vi "DialogAddDesignPattern.vi"(0 "ClassWriterNative":refnum<class "ClassWriterNative.lvclass">, 1 "ClassItemRefIn":refnum<vi>, 5 "error in (no error)":errorcluster) -> (14 "ClassWriterNative":refnum<class "ClassWriterNative.lvclass">, 15 "ClassItemRefOut":refnum<vi>, 16 "AddDesignPatternData":T1, 17 "Cancelled":bool, 19 "error out":errorcluster)   [LabVIEW 2020, in "ClassWriterNative.lvclass"]
uses:
  ClassWriterNative.lvclass
  Provider_BaseClassInterface/AddDesignPatternData.ctl
  Provider_BaseClassInterface/DesignPatternsData.ctl
  Common/LvClass_class/GDSLvClass_PlugIn.ctl
  Common/LvClass_class/GDSLvClass_PlugInTypes.ctl
  Provider_BaseClassInterface/BaseProvider_SubVIs/BaseProvider_DesignPatternsActions.ctl
  ClassWriterNative.lvclass/ClassWriterNative.ctl
panel:
  out "ProductPicture":picture
  out "TextError":string
  out "_Description":string caption="Description"
  in  "_DesignPatterns":string(tree) caption="Design Patterns"
  out "_ClassTemplateUsed":string caption="Class Template Used"
  out "_ClassProviderName":string caption="Class Provider Name"
  out "_ClassName":string caption="Class name"
  in  "_ShowContextHelp":bool
  in  "Help":bool
  in  "_Cancel":bool
  in  "_Next":bool
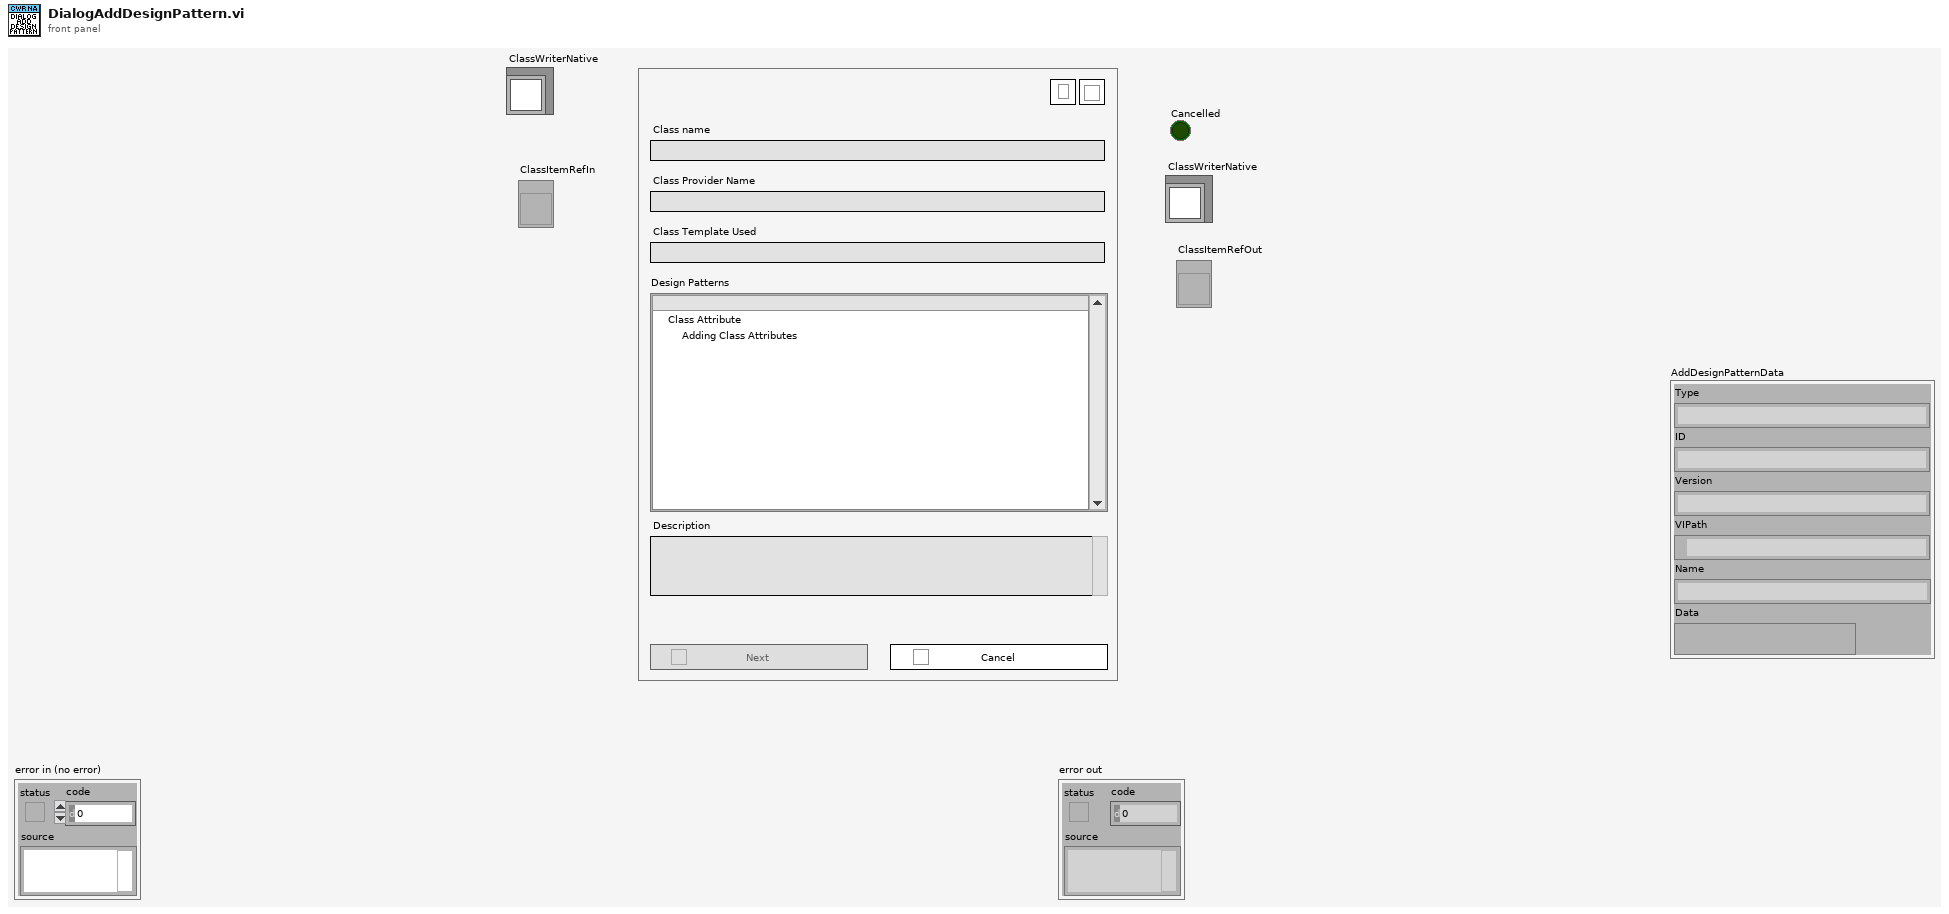
[diagram p1: front panel]
types:
  T1 = typedef "AddDesignPatternData.ctl" = cluster{"Type":string, "ID":string, "Version":string, "VIPath":path, "Name":string, "Data":variant}
  T2 = typedef "DesignPatternsData.ctl" = cluster{"Type":string, "Patterns":cluster{"ID":string, "Path":path, "Name":string, "Desc":string, "Version":string, "DependenciesID":string[], "OnlyOne":bool}[]}
  T3 = cluster{"Cancel":bool, "ClassProviderName":string, "ClassTemplateUsed":string, "DesignPatterns":T2[], "DataOut":variant, "PlugInVI":path, "DesignPatternID":string, "DesignPatternType":string, "PlugInIDs":string[], "DesignPatternVer":string, "Name":string}
  T4 = typedef "BaseProvider_DesignPatternsActions.ctl" = enum16{"AddPatternDialog", "GeneratePattern", "RemovePattern", "CreatePatternMethod", "UpdatePattern"}
  T5 = typedef "GDSLvClass_PlugIn.ctl" = cluster{"Type":T6, "ID":string, "Version":string, "Path":path, "Name":string, "Data":variant}
  T6 = typedef "GDSLvClass_PlugInTypes.ctl" = enum16{"DesignPattern", "MethodTypes"}
  T7 = typedef "GDSLvCLass_ClassSettingsType.ctl" = cluster{"ClassProviderName":string, "ClassTemplateUsed":string, "ClassTemplateVersion":string, "ClassDescription":string, "PlugIns":T5[], "ConnectorPanePattern":string}
  T8 = cluster{"ID":string, "Path":path, "Name":string, "Desc":string, "Version":string, "DependenciesID":string[], "OnlyOne":bool}[]
  T9 = cluster{"ID":string, "Path":path, "Name":string, "Desc":string, "Version":string, "DependenciesID":string[], "OnlyOne":bool}
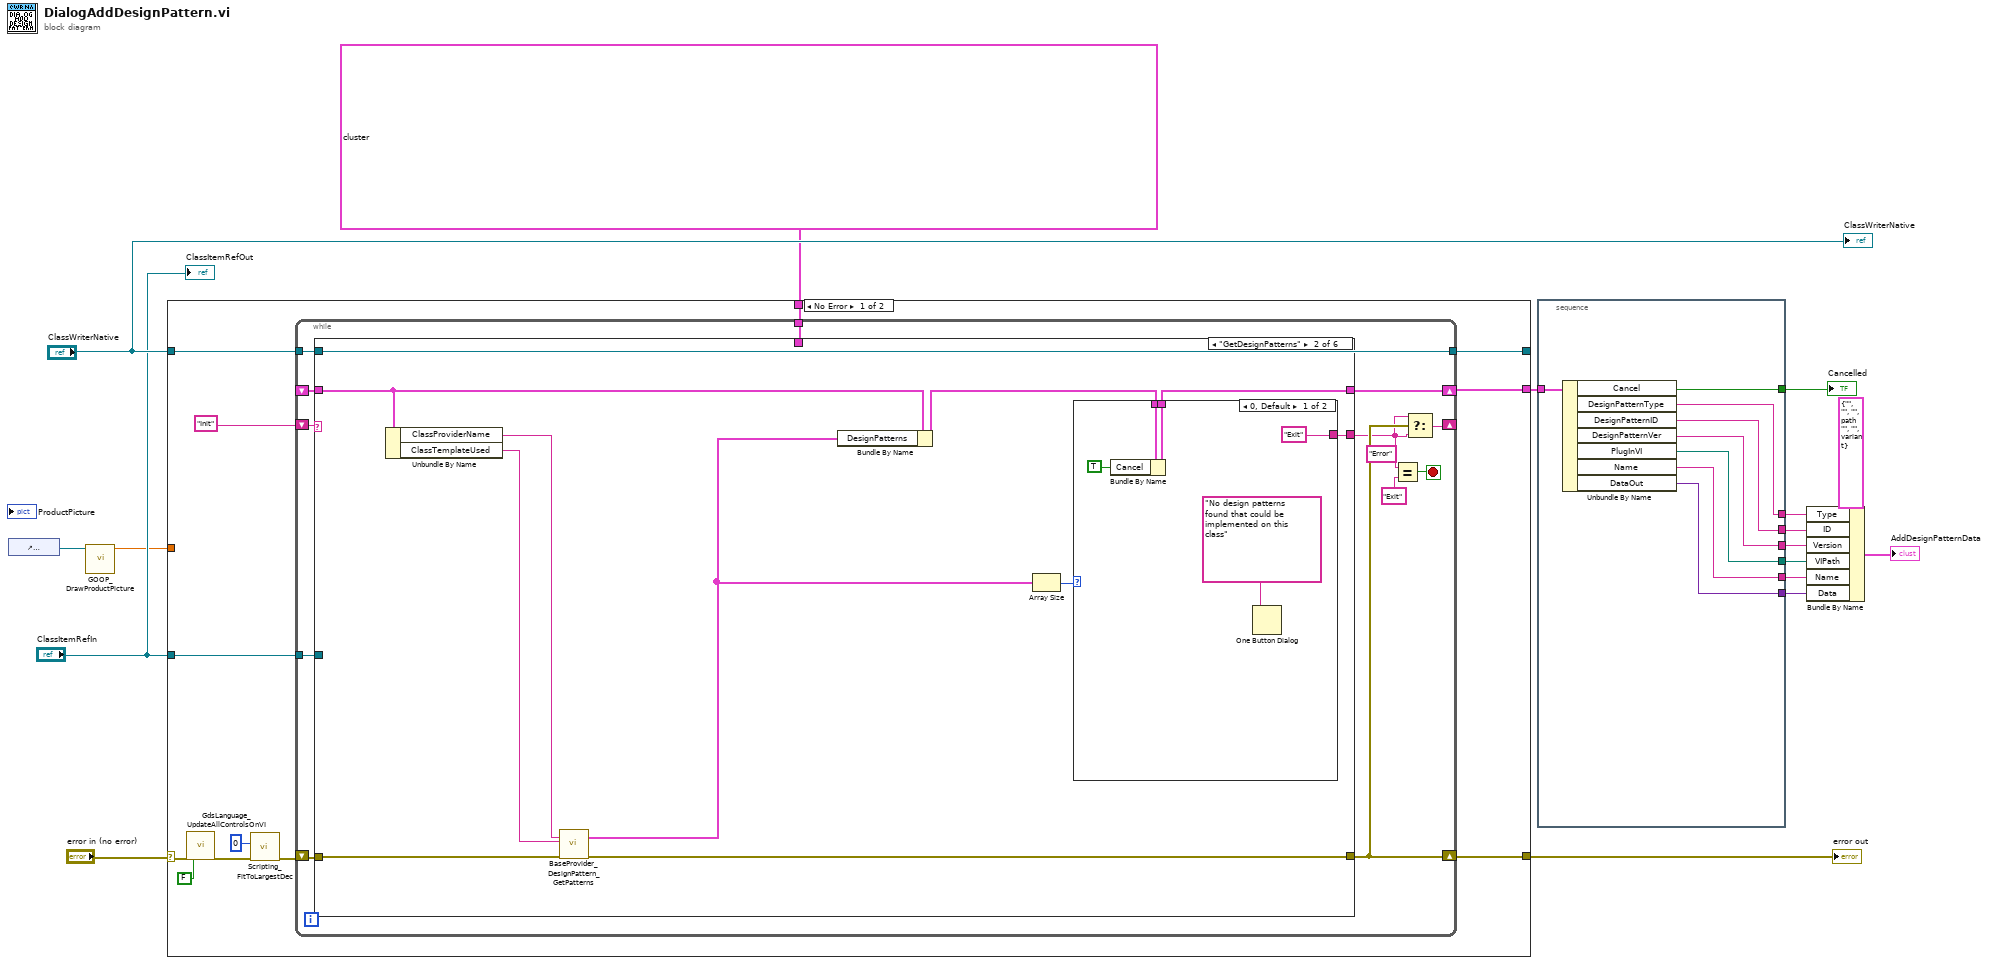
[diagram p0: block diagram]
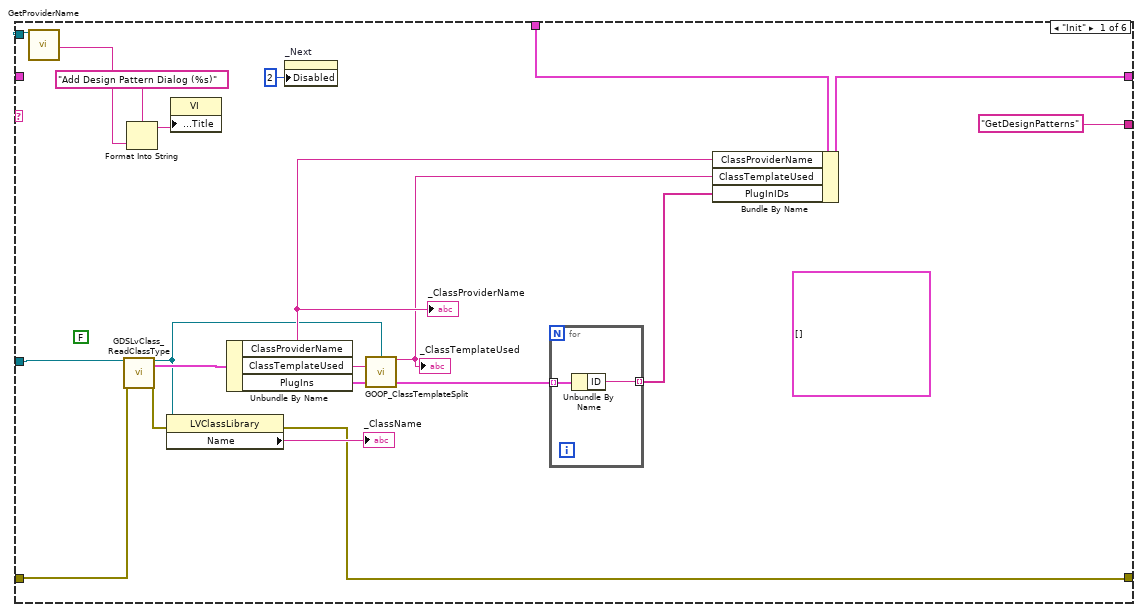
[diagram p2: hidden frame]
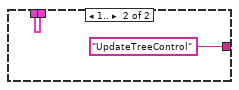
[diagram p3: hidden frame]
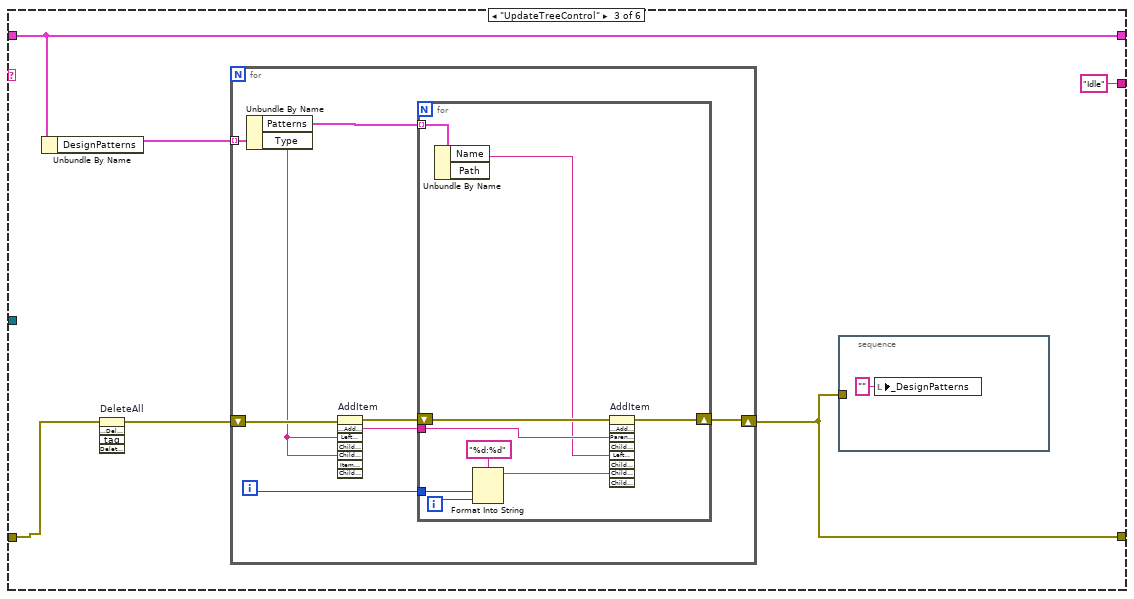
[diagram p4: hidden frame]
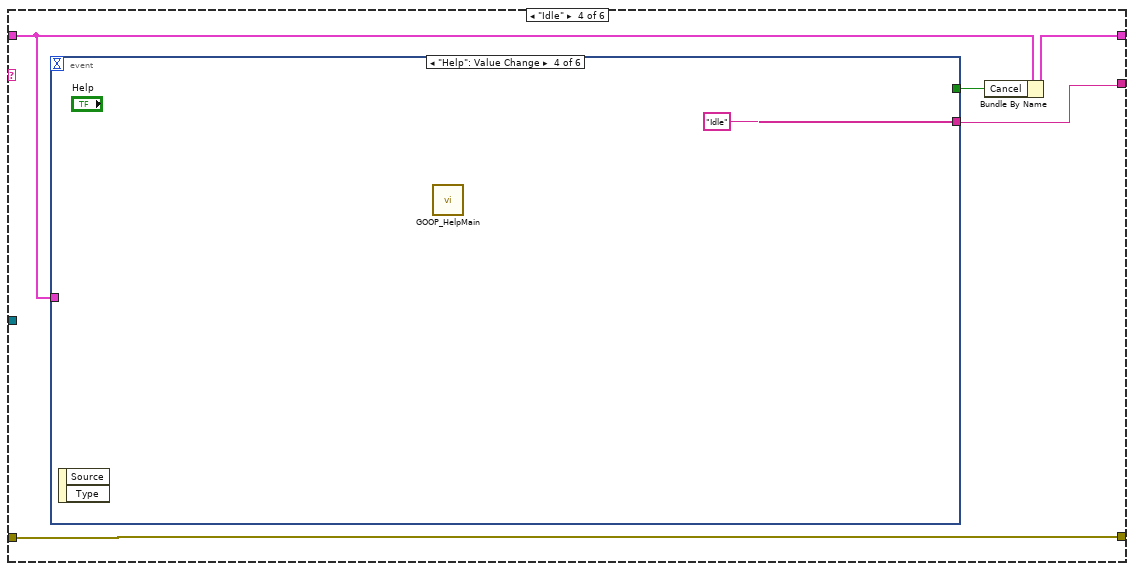
[diagram p5: hidden frame]
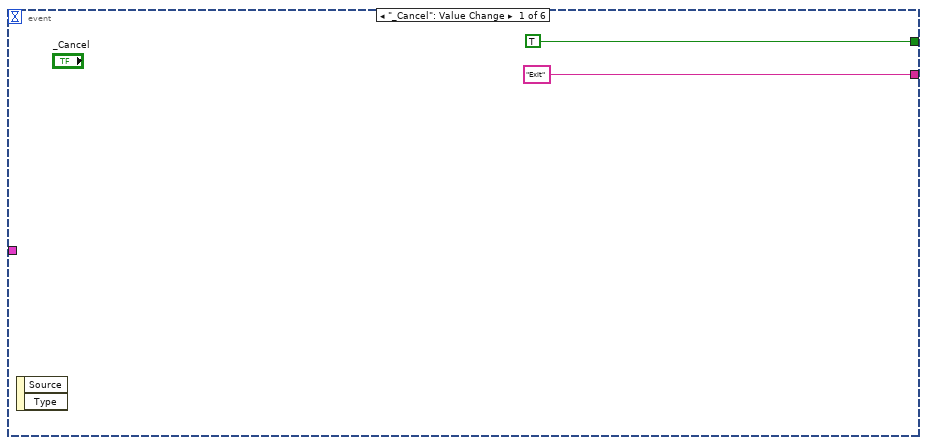
[diagram p6: hidden frame]
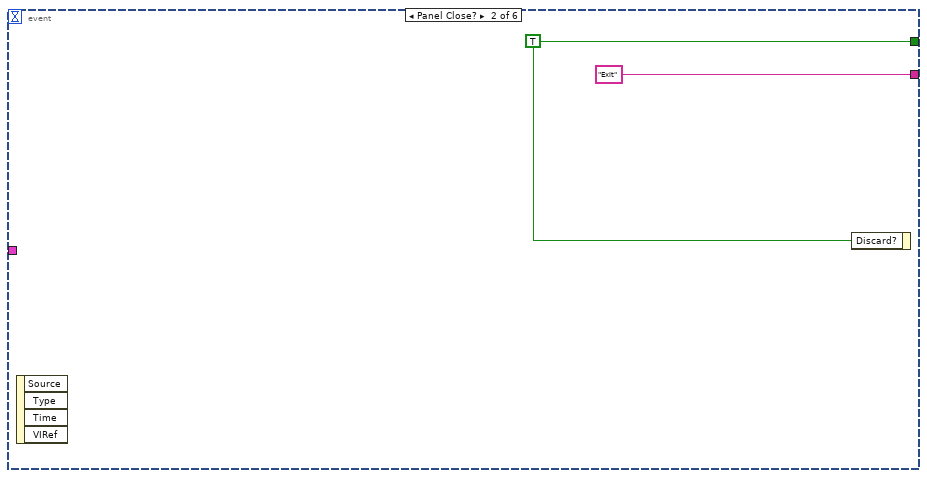
[diagram p7: hidden frame]
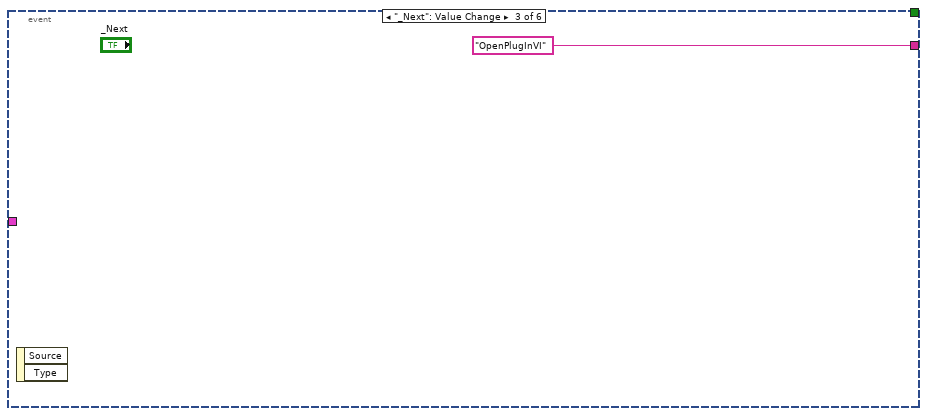
[diagram p8: hidden frame]
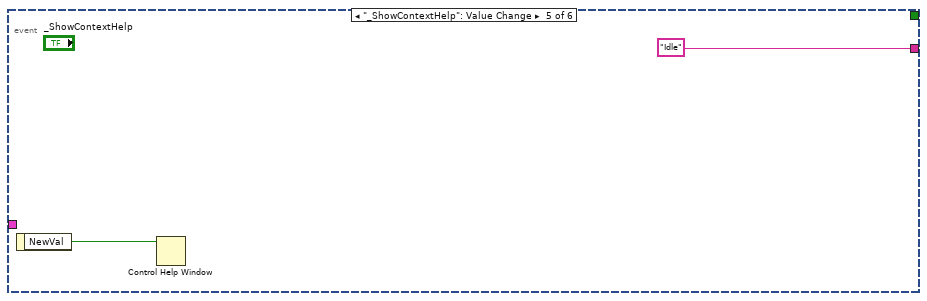
[diagram p9: hidden frame]
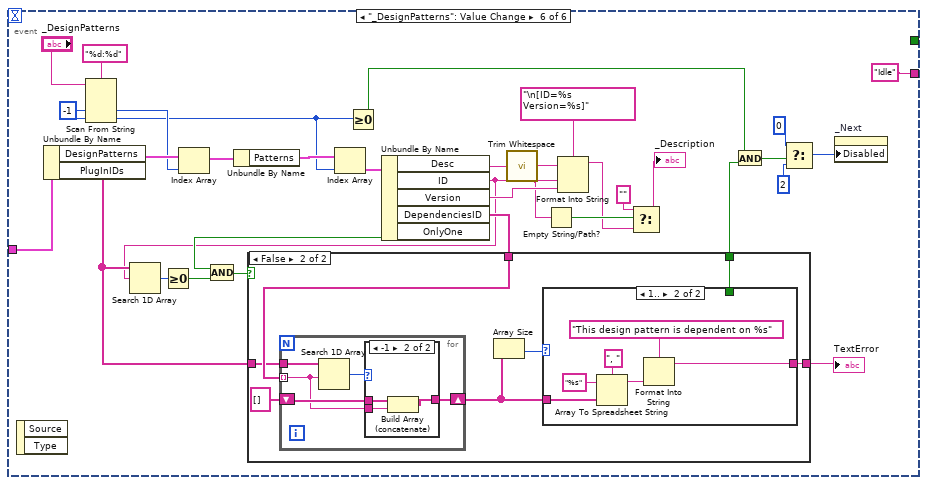
[diagram p10: hidden frame]
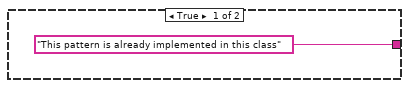
[diagram p11: hidden frame]
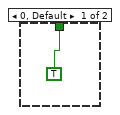
[diagram p12: hidden frame]
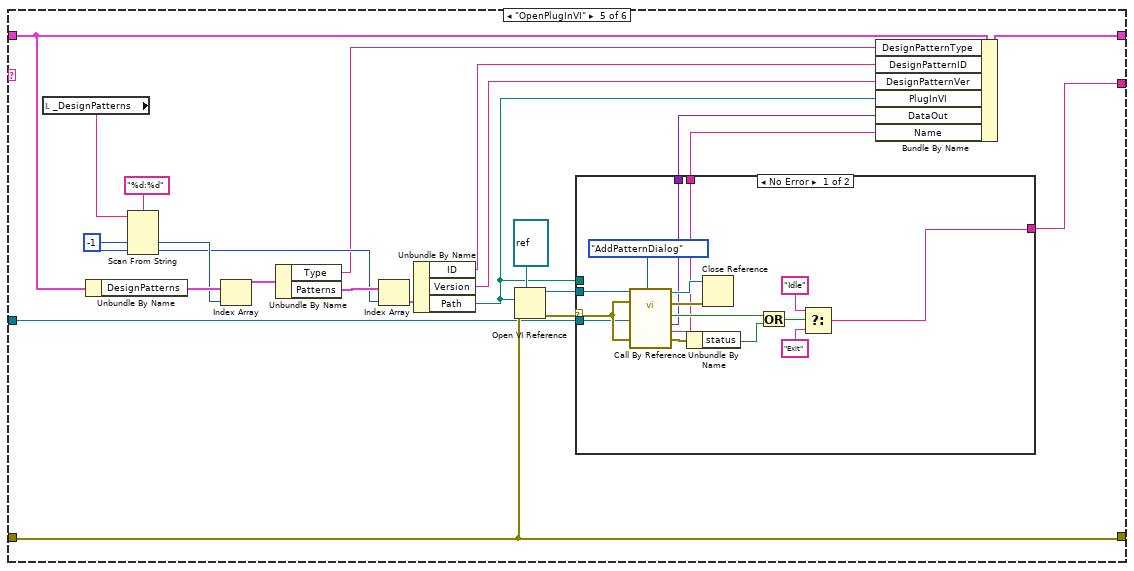
[diagram p14: hidden frame]
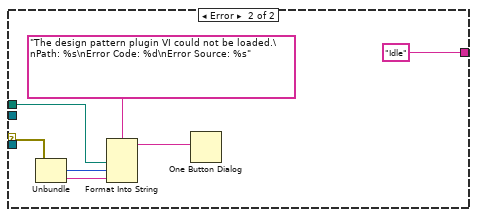
[diagram p15: hidden frame]
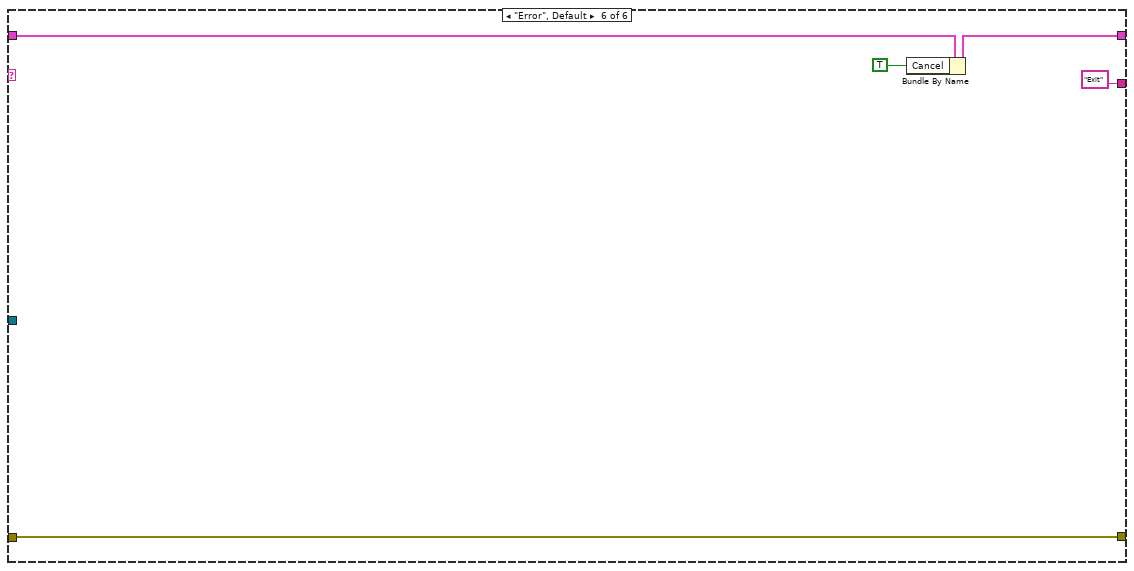
[diagram p16: hidden frame]
diagram:
  n1 = control-ref of="ProductPicture"() -> (w2:refnum<vi>)
  n2 = call "GOOP_DrawProductPicture.vi"("ProductPictureControl"=w2) -> ("Zoom Factor"=w1:sgl)  [unwired: 10 in]
  n3 = case shown="No Error" "error in (no error)" {
    selector: "error in (no error)" -> [w22 w227]
    tunnel: "ClassWriterNative" -> [w26 w226]
    tunnel: [w29 w227] -> w14
    tunnel: [w27 w226] -> _
    tunnel: T3 {"Cancel"=FALSE, "ClassProviderName"="", "ClassTemplateUsed"="", "DesignPatterns"=[], "DataOut"=variant, "PlugInVI"=path "", "DesignPatternID"="", "DesignPatternType"="", "PlugInIDs"=[], "DesignPatternVer"="", "Name"=""} ("output cluster") -> [w25 _]
    tunnel: "ClassItemRefIn" -> [w24 _]
    tunnel: [w23 _] -> w16
    tunnel: w1 -> [_ _]
    frame No Error {
      n4 = call "GdsLanguage_UpdateAllControlsOnVI.vi"("error in (no error)"=w22, "CreateLanguageFile(Use this to create a languageFile)"=FALSE) -> ("error out"=w19:errorcluster)  [unwired: 16 in, 1 out]
      n5 = call "Scripting_FitToLargestDec.vi"("error in (no error)"=w19, "border spacing (2 px)"=0) -> ("error out"=w18:errorcluster)  [unwired: 4 in, 1 out]
      n6 = while {
        shift-right: [w36] -> w29
        shift-left: w18 -> [w42]
        shift-right: [w35] -> _
        shift-left: "Init" -> [w39]
        shift-right: [w40] -> w23
        shift-left: _ -> [w41]
        tunnel: w26 -> [w32]
        tunnel: [w32] -> w27
        tunnel: w25 -> [w31]
        tunnel: w24 -> [w30]
        stop <- w37 stop-if-true
        n7 = case shown="\"GetDesignPatterns\"" w39 {
          tunnel: w41 -> [_ w67 w86 w106 w188 w223]
          tunnel: [w49 w65 w86 w108 w186 w222] -> w40
          tunnel: w42 -> [w56 w72 w85 w110 w185 w224]
          tunnel: [w52 w69 w82 w110 w185 w224] -> w36
          tunnel: w32 -> [w58 _ _ _ _ _]
          tunnel: ["GetDesignPatterns" w74 "Idle" w109 w183 "Exit"] -> w34
          tunnel: w31 -> [w50 _ _ _ _ _]
          tunnel: w30 -> [w57 _ _ _ w180 _]
          frame "Init" {
            (unwired) T5[] [] ("PlugIns")
            (unwired) FALSE ("Visible")
            n8 = call-dynamic "GetProviderName.vi"("ClassWriterNative in"=w58) -> ("TranslatedProviderName"=w43:string)  [unwired: 15 in, 3 out]
            n9 = call "GDSLvClass_ReadClassType.vi"("Class Refnum In"=w57, "error in (no error)"=w56) -> ("Class Refnum Out"=w44:refnum<vi>, "ClassSettings"=w55:T7, "error out"=w53:errorcluster)  [unwired: 15 in]
            n10 = Format Into String(format string="Add Design Pattern Dialog (%s)", w43) -> (resulting string=w60:string)  [unwired: 2 in, 1 out]
            n11 = property class="LVClassLibrary"(reference=w44, error in=w53) -> (error out=w52:errorcluster, "Name"=→"_ClassName":string)  [unwired: 1 out]
            n12 = property class="VI"("Front Panel.Title"=w60) -> ()  [unwired: 2 in, 2 out]
            n13 = Unbundle By Name(w55) -> ("ClassProviderName"=w51:string, "ClassTemplateUsed"=w46:string, "PlugIns"=w48:T5[])
            "_ClassProviderName" <- w51
            n14 = property on="_Next" class="Bool"("Disabled"=u8 2) -> ()  [unwired: 2 in, 2 out]
            n15 = call "GOOP_ClassTemplateSplit.vi"("ClassItemRefIn"=w44, "FullClassTemplate"=w46) -> ("StandardTemplate"=w45:string)  [unwired: 12 in, 1 out]
            "_ClassTemplateUsed" <- w45
            n16 = for {
              tunnel: w48 -> [w64] mode=indexing
              tunnel: [w63] -> w47 mode=indexing
              n17 = Unbundle By Name(w64) -> ("ID"=w63:string)
            }
            n18 = Bundle By Name(cluster=w50, "ClassProviderName"=w51, "ClassTemplateUsed"=w45, "PlugInIDs"=w47) -> (w49:T3)
          }
          frame "GetDesignPatterns" {
            n19 = Unbundle By Name(w67) -> ("ClassProviderName"=w71:string, "ClassTemplateUsed"=w70:string)
            n20 = call "BaseProvider_DesignPattern_GetPatterns.vi"("FilterOnProviders(Ignored If Empty)"=w71, "FilterOnTemplate(Ignored If Empty)"=w70, "error in (no error)"=w72) -> ("DesignPatterns"=w68:T2[], "error out"=w69:errorcluster)  [unwired: 15 in]
            n21 = Bundle By Name(cluster=w67, "DesignPatterns"=w68) -> (w66:T3)
            n22 = Array Size(array=w68) -> (size(s)=w73:i32)
            n23 = case shown="0, Default" w73 {
              tunnel: ["Exit" "UpdateTreeControl"] -> w74
              tunnel: w66 -> [w77 w80]
              tunnel: [w76 w80] -> w65
              frame 0, Default {
                n24 = Bundle By Name(cluster=w77, "Cancel"=TRUE) -> (w76:T3)
                n25 = One Button Dialog(message="No design patterns found that could be implemented on this class" ("format string")) -> ()  [unwired: 1 in, 1 out]
              }
              frame 1.. {
              }
            }
          }
          frame "UpdateTreeControl" {
            n26 = Unbundle By Name(w86) -> ("DesignPatterns"=w83:T2[])
            n27 = invoke on="DeleteAll" class="Tree (strict)" method="Edit Tree Items.Delete"(error in=w85) -> (error out=w84:errorcluster)  [unwired: 4 in, 4 out]
            n28 = for {
              shift-right: [w89] -> w82
              shift-left: w84 -> [w96]
              tunnel: w83 -> [w95] mode=indexing
              i -> [w90]
              n29 = Unbundle By Name(w95) -> ("Patterns"=w91:T8, "Type"=w92:string)
              n30 = invoke on="AddItem" class="Tree (strict)" method="Edit Tree Items.Add Item to End"(error in=w96, "Left Cell"=w92, "Child Tag"=w92) -> (error out=w94:errorcluster, "Edit Tree Items:Add Item to End"=w93:string)  [unwired: 5 in, 6 out]
              n31 = for {
                shift-right: [w97] -> w89
                shift-left: w94 -> [w104]
                tunnel: w93 -> [w105]
                tunnel: w91 -> [w103] mode=indexing
                tunnel: w90 -> [w100]
                i -> [w99]
                n32 = Unbundle By Name(w103) -> ("Name"=w102:string)  [unwired: 1 out]
                n33 = Format Into String(format string="%d:%d", w100, w99) -> (resulting string=w98:string)  [unwired: 2 in, 1 out]
                n34 = invoke on="AddItem" class="Tree (strict)" method="Edit Tree Items.Add Item"(error in=w104, "Parent Tag"=w105, "Left Cell"=w102, "Child Tag"=w98) -> (error out=w97:errorcluster)  [unwired: 5 in, 8 out]
              }
            }
            n35 = stacked-sequence {
              tunnel: w82 -> [_]
              frame #0 {
                n36 = local write "_DesignPatterns"("" ("_DesignPatterns")) -> ()
              }
            }
          }
          frame "Idle" {
            n37 = event shown="[3] \"Help\": Value Change" {
              selector: _ -> [_ _ _ _ _ _]
              dyn-events: _ -> [_ _ _ _ _ _]
              timeout: _ -> [_ _ _ _ _ _]
              tunnel: ["Exit" "Exit" "OpenPlugInVI" "Idle" "Idle" "Idle"] -> w109
              tunnel: [TRUE w113 _ _ _ _] -> w107
              tunnel: w106 -> [_ _ _ _ _ w150]
              event "_Cancel": Value Change {
                n38 = event-data() -> ()  [unwired: 1 in, 2 out]
              }
              event Panel Close? {
                w113 = TRUE
                n39 = event-data() -> ()  [unwired: 1 in, 4 out]
                n40 = event-data("Discard?"=w113) -> ()  [unwired: 1 in, 1 out]
              }
              event "_Next": Value Change {
                n41 = event-data() -> ()  [unwired: 1 in, 2 out]
              }
              event "Help": Value Change {
                n42 = event-data() -> ()  [unwired: 1 in, 2 out]
                n43 = call "GOOP_HelpMain.vi"() -> ()  [unwired: 12 in]
              }
              event "_ShowContextHelp": Value Change {
                n44 = event-data() -> ("NewVal"=w117:bool)  [unwired: 1 in]
                n45 = Control Help Window(1:w117) -> ()  [unwired: 1 in]
              }
              event "_DesignPatterns": Value Change {
                w138 = -1 ("default value 1")
                n46 = event-data() -> ()  [unwired: 1 in, 2 out]
                n47 = Unbundle By Name(w150) -> ("DesignPatterns"=w149:T2[], "PlugInIDs"=w128:string[])
                n48 = Scan From String(format string="%d:%d", input string="_DesignPatterns", default 1=w138, default 2=w138) -> (output 1=w148:i32, output 2=w145:i32)  [unwired: 2 in, 3 out]
                n49 = Index Array(array=w149, index=w148) -> (element=w147:T2)
                n50 = Unbundle By Name(w147) -> ("Patterns"=w146:T8)
                n51 = Index Array(array=w146, index=w145) -> (element=w143:T9)
                n52 = Greater Or Equal To 0?(x=w145) -> (x >= 0?=w133:bool)
                n53 = Unbundle By Name(w143) -> ("Desc"=w137:string, "ID"=w122:string, "Version"=w130:string, "DependenciesID"=w135:string[], "OnlyOne"=w124:bool)
                n54 = Search 1D Array(1D array=w128, element=w122) -> (index of element=w127:i32)  [unwired: 1 in]
                n55 = Greater Or Equal To 0?(x=w127) -> (x >= 0?=w126:bool)
                n56 = Compound Arithmetic op=AND(w124, w126) -> (w125:bool)
                n57 = case shown="False" w125 {
                  tunnel: w135 -> [_ w159]
                  tunnel: ["This pattern is already implemented in this class" w156] -> w134
                  tunnel: [_ w154] -> w131
                  tunnel: w128 -> [_ w153]
                  frame True {
                  }
                  frame False {
                    n58 = for {
                      tunnel: w159 -> [w168] mode=indexing
                      tunnel: w153 -> [w171]
                      shift-right: [w167] -> w157
                      shift-left: string[] [] -> [w169]
                      n59 = Search 1D Array(1D array=w171, element=w168) -> (index of element=w170:i32)  [unwired: 1 in]
                      n60 = case shown="-1" w170 {
                        tunnel: w169 -> [w172 w175]
                        tunnel: w168 -> [_ w174]
                        tunnel: [w172 w173] -> w167
                        frame Default {
                        }
                        frame -1 {
                          n61 = Build Array (concatenate)(w175, w174) -> (w173:string[])
                        }
                      }
                    }
                    n62 = Array Size(array=w157) -> (size(s)=w155:i32)
                    n63 = case shown="1.." w155 {
                      tunnel: w157 -> [_ w166]
                      tunnel: [_ w161] -> w156
                      tunnel: [TRUE _] -> w154
                      frame 0, Default {
                      }
                      frame 1.. {
                        n64 = Array To Spreadsheet String(delimiter (Tab)=", ", array=w166, 3:"%s" ("format string")) -> (spreadsheet string=w163:string)
                        n65 = Format Into String(format string="This design pattern is dependent on %s", w163) -> (resulting string=w161:string)  [unwired: 2 in, 1 out]
                      }
                    }
                  }
                }
                "TextError" <- w134
                n66 = call <vilib>:"Trim Whitespace.vi"("string"=w137) -> ("trimmed string"=w136:string)  [unwired: 1 in]
                n67 = Empty String/Path?(string/path=w122) -> (empty?=w123:bool)
                n68 = Format Into String(format string="\n[ID=%s Version=%s]", initial string=w136, w122, w130) -> (resulting string=w121:string)  [unwired: 1 in, 1 out]
                n69 = Select(t="" ("ID"), s=w123, f=w121) -> (s? t:f=→"_Description":string)
                n70 = And(x=w133, y=w131) -> (x .and. y?=w132:bool)
                n71 = Select(t=u8 0, s=w132, f=u8 2 ("Disabled")) -> (s? t:f=w140:u8)
                n72 = property on="_Next" class="Bool"("Disabled"=w140) -> ()  [unwired: 2 in, 2 out]
              }
            }
            n73 = Bundle By Name(cluster=w106, "Cancel"=w107) -> (w108:T3)
          }
          frame "OpenPlugInVI" {
            w181 = -1 ("default value 1")
            n74 = local read "_DesignPatterns"() -> (w191:string)
            n75 = Unbundle By Name(w188) -> ("DesignPatterns"=w197:T2[])
            n76 = Scan From String(format string="%d:%d", input string=w191, default 1=w181, default 2=w181) -> (output 1=w196:i32, output 2=w193:i32)  [unwired: 2 in, 3 out]
            n77 = Index Array(array=w197, index=w196) -> (element=w195:T2)
            n78 = Unbundle By Name(w195) -> ("Type"=w179:string, "Patterns"=w194:T8)
            n79 = Index Array(array=w194, index=w193) -> (element=w192:T9)
            n80 = Unbundle By Name(w192) -> ("ID"=w178:string, "Version"=w177:string, "Path"=w182:path)
            n81 = Open VI Reference(type specifier VI Refnum (for type only)=refnum<vi> refnum, vi path=w182, error in (no error)=w185) -> (vi reference=w189:refnum<vi>, error out=w184:errorcluster)  [unwired: 3 in]
            n82 = case shown="No Error" w184 {
              selector: w184 -> [w205 w218]
              tunnel: w189 -> [w213 _]
              tunnel: [w206 _] -> w187
              tunnel: w182 -> [_ w215]
              tunnel: [w203 "Idle"] -> w183
              tunnel: w180 -> [w201 _]
              tunnel: [w199 _] -> w176
              frame No Error {
                n83 = call-by-ref "?"(reference=w213, error in=w205, "Action"=BaseProvider_DesignPatternsActions."AddPatternDialog", 8:"error in (no error)"=w205, "ClassRefToActOn"=w201) -> (reference out=w208:refnum<vi>, error out=w209:errorcluster, 0:"error out"=w212:errorcluster, "Name"=w199:string, "DataOut"=w206:variant, "Cancelled"=w211:bool)  [unwired: 5 in]
                n84 = Unbundle By Name(w212) -> ("status"=w210:bool)
                n85 = Close Reference(reference=w208, error in (no error)=w209) -> ()  [unwired: 1 out]
                n86 = Or(x=w211, y=w210) -> (x .or. y?=w207:bool)
                n87 = Select(t="Idle", s=w207, f="Exit") -> (s? t:f=w203:string)
              }
              frame Error {
                n88 = Unbundle(w218) -> ("code"=w217:i32, "source"=w216:string)  [unwired: 1 out]
                n89 = Format Into String(format string="The design pattern plugin VI could not be loaded.\nPath: %s\nError Code: %d\nError Source: %s" ("message"), w215, w217, w216) -> (resulting string=w219:string)  [unwired: 2 in, 1 out]
                n90 = One Button Dialog(message=w219) -> ()  [unwired: 1 in, 1 out]
              }
            }
            n91 = Bundle By Name(cluster=w188, "DesignPatternType"=w179, "DesignPatternID"=w178, "DesignPatternVer"=w177, "PlugInVI"=w182, "DataOut"=w187, "Name"=w176) -> (w186:T3)
          }
          frame "Error", Default {
            n92 = Bundle By Name(cluster=w223, "Cancel"=TRUE) -> (w222:T3)
          }
        }
        n93 = Equal?(x=w34, y="Exit") -> (x = y?=w37:bool)
        n94 = Select(t="Error", s=w36, f=w34) -> (s? t:f=w35:string)
      }
    }
    frame Error {
    }
  }
  "error out" <- w14
  n95 = stacked-sequence {
    tunnel: w16 -> [w235]
    tunnel: [w234] -> w15
    tunnel: [w233] -> w7
    tunnel: [w232] -> w8
    tunnel: [w231] -> w6
    tunnel: [w230] -> w5
    tunnel: [w229] -> w4
    tunnel: [w228] -> w3
    frame #0 {
      n96 = Unbundle By Name(w235) -> ("Cancel"=w234:bool, "DesignPatternType"=w230:string, "DesignPatternID"=w231:string, "DesignPatternVer"=w229:string, "PlugInVI"=w233:path, "Name"=w228:string, "DataOut"=w232:variant)
    }
  }
  "Cancelled" <- w15
  n97 = Bundle By Name(cluster=T1 {"Type"="", "ID"="", "Version"="", "VIPath"=path "", "Name"="", "Data"=variant} ("AddDesignPatternData"), "Type"=w5, "ID"=w6, "Version"=w4, "VIPath"=w7, "Name"=w3, "Data"=w8) -> (→"AddDesignPatternData":T1)
  "ClassWriterNative" <- "ClassWriterNative"
  "ClassItemRefOut" <- "ClassItemRefIn"
